vi "Destroy Test Suite.vi"(8 "error in (no error)":errorcluster, 11 "Test Suite in":refnum<class "Test Suite.lvclass">) -> (0 "error out":errorcluster, 3 "Test Suite Results":refnum<class "Test Result.lvclass">)   [LabVIEW 2020, in "Caraya.lvlib" / "Test Suite.lvclass"]
doc: "Destroys a test suite."
uses:
  Test Suite.lvclass
  Test Result/Test Result.lvclass
  Test Suite.lvclass/Test Suite.ctl
  Test Assert Factory/Test Assert Factory.lvclass/Test Assert Factory.ctl
  Properties.Suite/Properties.Suite.lvclass/Properties.Suite.ctl
  Test Assert Factory/Test Assert Factory.lvclass
  Assert Factory Manager/Assert Factory Manager.lvclass
  Properties.Suite/Properties.Suite.lvclass
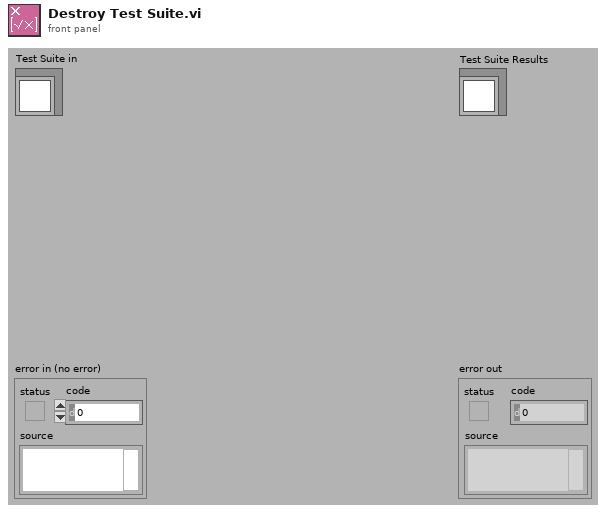
[diagram p1: front panel]
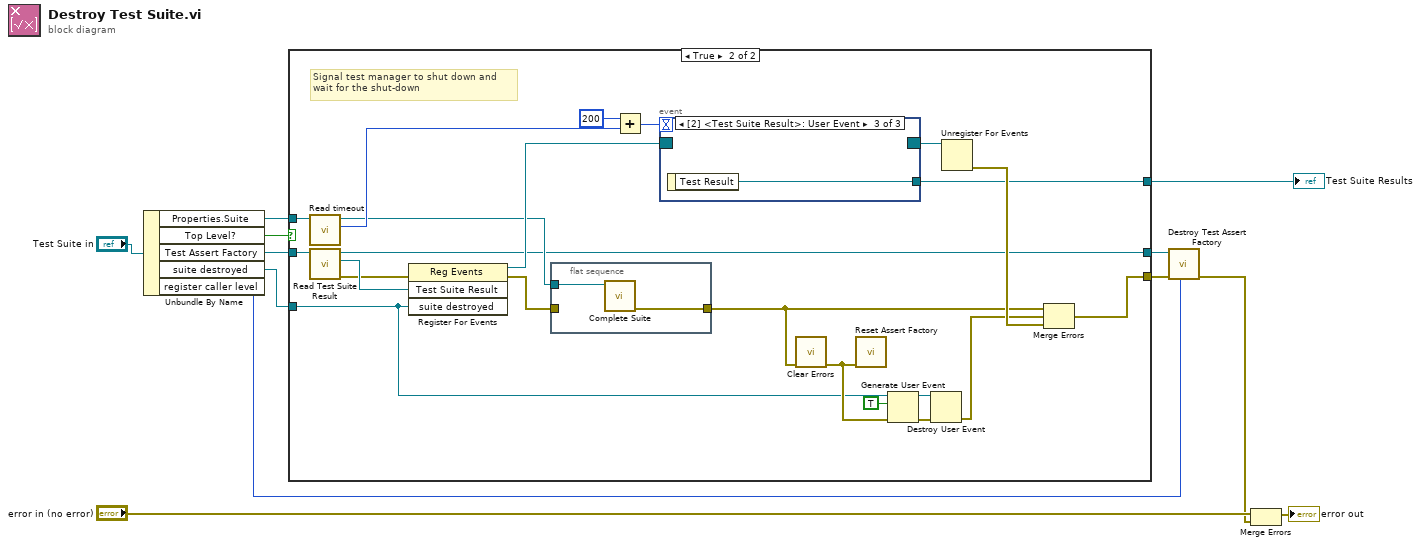
[diagram p0: block diagram]
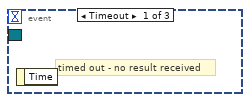
[diagram p3: hidden frame]
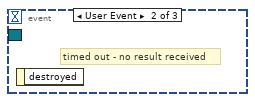
[diagram p4: hidden frame]
diagram:
  n1 = Unbundle By Name("Test Suite in") -> ("Properties.Suite"=w2:refnum<class "Properties.Suite.lvclass">, "Top Level?"=w10:bool, "Test Assert Factory"=w9:refnum<class "Test Assert Factory.lvclass">, "suite destroyed"=w3:refnum<user-event>, "register caller level"=w1:i32)
  n2 = case shown="True" w10 {
    tunnel: [_ w35] -> w8
    tunnel: w9 -> [w13 w34]
    tunnel: [w13 w14] -> w6
    tunnel: [_ w23] -> w4
    tunnel: w3 -> [_ w19]
    tunnel: w2 -> [_ w22]
    frame False {
    }
    frame True {
      # "Signal test manager to shut down and \nwait for the shut-down"
      n3 = call "Read timeout.vi"("Properties.Suite in"=w22) -> ("timeout"=w21:i32, "Properties.Suite out"=w18:refnum<class "Properties.Suite.lvclass">)  [unwired: 9 in]
      n4 = call "Read Test Suite Result.vi"("Test Assert Factory in"=w34) -> ("error out"=w32:errorcluster, "Test Suite Result"=w33:refnum<user-event>, "Test Assert Factory out"=w14:refnum<class "Test Assert Factory.lvclass">)  [unwired: 8 in]
      n5 = register-events(error in=w32, w33, w19) -> (reference out=w28:refnum<event-registration>, error out=w17:errorcluster)  [unwired: 1 in]
      n6 = flat-sequence {
        tunnel: w18 -> [w37]
        tunnel: w17 -> [_]
        tunnel: [w36] -> w15
        frame #0 {
          n7 = call "Complete Suite.vi"("Properties.Suite in"=w37) -> ("Test Suite Error"=w36:errorcluster)  [unwired: 9 in, 1 out]
        }
      }
      n8 = Add(x=200, y=w21) -> (x+y=w27:i32)
      n9 = event shown="[2] <Test Suite Result>: User Event" {
        selector: w28 -> [_ _ _]
        dyn-events: [_ _ _] -> w25
        timeout: w27 -> [_ _ _]
        tunnel: [_ _ w38] -> w23
        event Timeout {
          # "timed out - no result received"
          n10 = event-data() -> ()  [unwired: 1 in, 1 out]
        }
        event User Event {
          # "timed out - no result received"
          n11 = event-data() -> ()  [unwired: 1 in, 1 out]
        }
        event User Event {
          n12 = event-data() -> ("Test Result"=w38:refnum<class "Test Result.lvclass">)  [unwired: 1 in]
        }
      }
      n13 = call <vilib>:"Clear Errors.vi"("error in (no error)"=w15) -> ("error out"=w20:errorcluster)  [unwired: 5 in, 1 out]
      n14 = call "Reset Assert Factory.vi"("error in (no error)"=w20) -> ()  [unwired: 10 in, 1 out]
      n15 = Generate User Event(user event=w19, event data cluster=TRUE ("event data"), error in=w20) -> (user event out=w29:refnum<user-event>, error out=w30:errorcluster)  [unwired: 1 in]
      n16 = Destroy User Event(user event=w29, error in=w30) -> (error out=w16:errorcluster)
      n17 = Unregister For Events(event registration refnum=w25) -> (error out=w24:errorcluster)  [unwired: 1 in]
      n18 = Merge Errors(w15, w16, w24) -> (w35:errorcluster)
    }
  }
  "Test Suite Results" <- w4
  n19 = call-dynamic "Destroy Test Assert Factory.vi"("register caller level (0)"=w1, "error in (no error)"=w8, "Test Assert Factory in"=w6) -> ("error out"=w7:errorcluster)  [unwired: 8 in]
  n20 = Merge Errors("error in (no error)", w7) -> (→"error out":errorcluster)
